vi "GPIB_SR400.vi"(4 "Tset setting":dbl, 5 "N per point":i32, 6 "x":dbl) -> (0 "Array":string[](array[string]), 3 "x/y":dbl)   [LabVIEW 2024]
uses:
  <vilib>/Utility/error.llb/Trim Whitespace One-Sided.vi
  GPIB_Address.vi
panel:
  in  "Boolean":bool
  out "output array":string[](array[string])
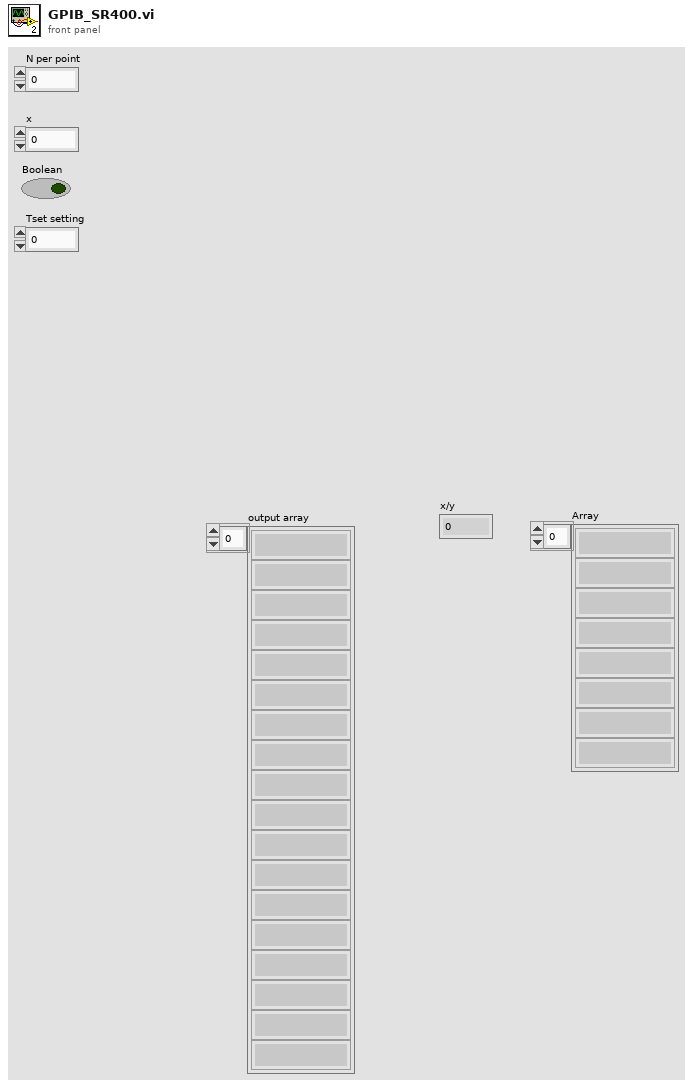
[diagram p1: front panel]
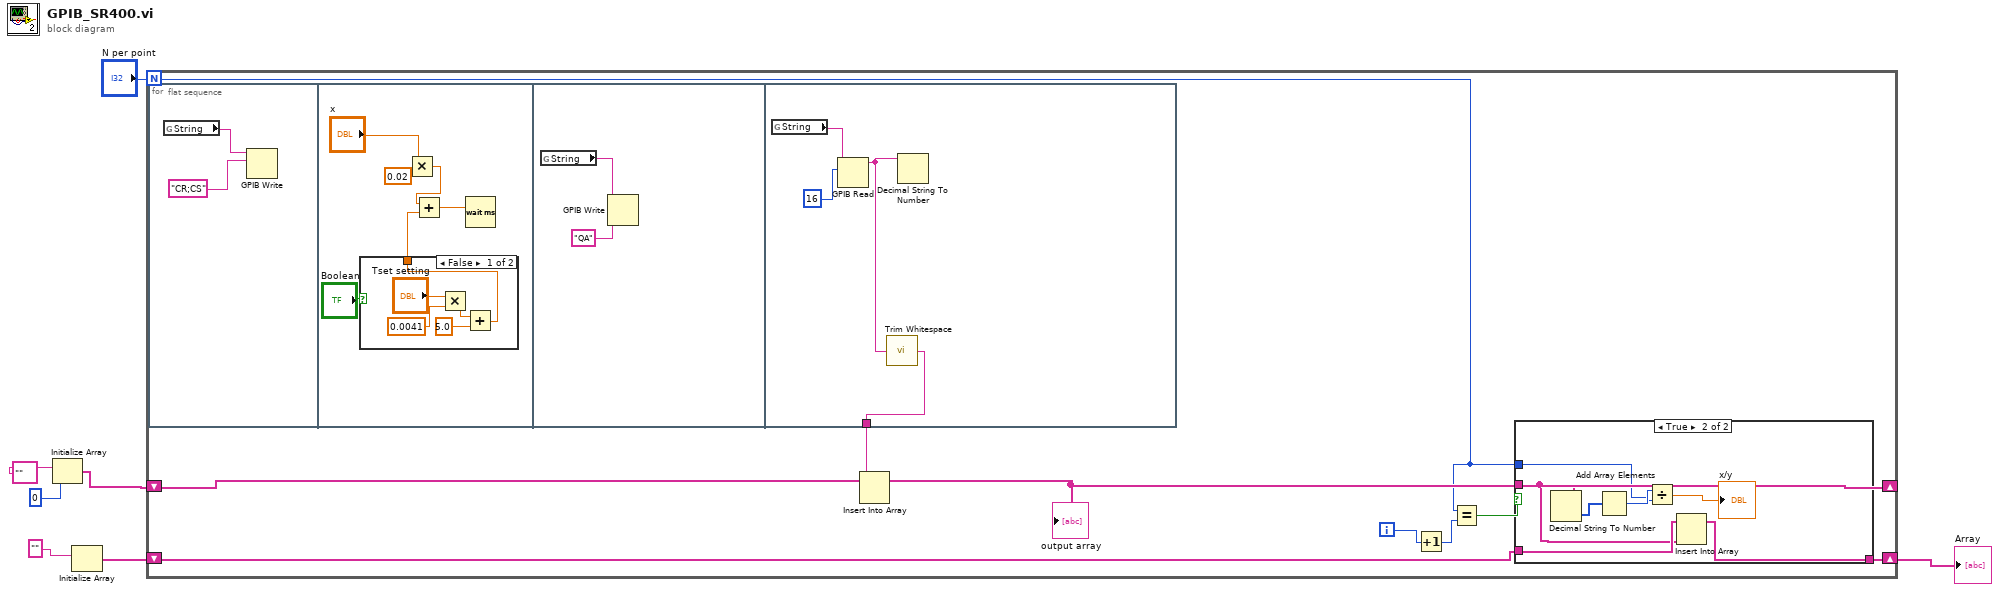
[diagram p0: block diagram]
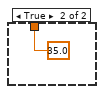
[diagram p3: hidden frame]
diagram:
  n1 = Initialize Array("", 0 ("dimension size")) -> (w6:string[])
  n2 = Initialize Array("") -> (w2:string[])  [unwired: 1 in]
  n3 = for {
    N: "N per point" -> [w12]
    shift-right: [w13] -> _
    shift-left: w6 -> [w16]
    shift-right: [w9] -> w1
    shift-left: w2 -> [w8]
    i -> [w10]
    n4 = flat-sequence {
      tunnel: [w42] -> w15
      frame #0 {
        n5 = global read "GPIB_Address.vi" "String"() -> (w24:string)
        n6 = GPIB Write(0:w24, 1:"CR;CS" ("data")) -> ()  [unwired: 3 in, 2 out]
      }
      frame #1 {
        n7 = case shown="False" "Boolean" {
          tunnel: [w32 35.0] -> w27
          frame False {
            n8 = Multiply(x="Tset setting", y=0.0041) -> (x*y=w34:dbl)
            n9 = Add(x=w34, y=5.0) -> (x+y=w32:dbl)
          }
          frame True {
          }
        }
        n10 = Multiply(x="x", y=0.02) -> (x*y=w28:dbl)
        n11 = Add(x=w28, y=w27) -> (x+y=w29:dbl)
        n12 = Wait (ms)(milliseconds to wait=w29) -> ()  [unwired: 1 out]
      }
      frame #2 {
        n13 = global read "GPIB_Address.vi" "String"() -> (w38:string)
        n14 = GPIB Write(0:w38, 1:"QA" ("data")) -> ()  [unwired: 3 in, 2 out]
      }
      frame #3 {
        n15 = global read "GPIB_Address.vi" "String"() -> (w40:string)
        n16 = GPIB Read(0:w40, 1:16 ("byte count")) -> (5:w41:string)  [unwired: 3 in, 2 out]
        n17 = call <vilib>:"Trim Whitespace.vi"("string"=w41) -> ("trimmed string"=w42:string)  [unwired: 1 in]
        n18 = Decimal String To Number(string=w41) -> ()  [unwired: 2 in, 2 out]
      }
    }
    n19 = Insert Into Array(array=w16, new element=w15) -> (w13:string[])  [unwired: 1 in]
    "output array" <- w13
    n20 = Increment(x=w10) -> (x+1=w11:i32)
    n21 = Equal?(x=w12, y=w11) -> (x = y?=w14:bool)
    n22 = case shown="True" w14 {
      tunnel: w13 -> [_ w18]
      tunnel: w12 -> [_ w21]
      tunnel: [_ w17] -> w9
      tunnel: w8 -> [_ w19]
      frame False {
      }
      frame True {
        n23 = Decimal String To Number(string=w18) -> (number=w23:i32[])  [unwired: 2 in, 1 out]
        n24 = Add Array Elements(numeric array=w23) -> (sum=w22:i32)
        n25 = Divide(x=w22, y=w21) -> (x/y=→"x/y":dbl)
        n26 = Insert Into Array(array=w19, new element=w18) -> (w17:string[])  [unwired: 1 in]
      }
    }
  }
  "Array" <- w1
